vi "libssh2_userauth_password_ex.vi"(7 "passwd_change_cb":u64, 8 "error in (no error)":errorcluster, 9 "password":string, 10 "username":string, 11 "session":T1) -> (0 "error out":errorcluster)   [LabVIEW 2017, in "libssh2.lvlib"]
doc: "Authenticate a session using a password with a custom password change callback."
uses:
  libssh2.lvlib
  Session Refnum.ctl
  Not A Session.vi
  <vilib>/Utility/error.llb/Error Cluster From Error Code.vi
  Global Settings.vi
  Read Session Refnum.vi
  <vilib>/Utility/semaphor.llb/Acquire Semaphore.vi
  <vilib>/Utility/semaphor.llb/Release Semaphore.vi
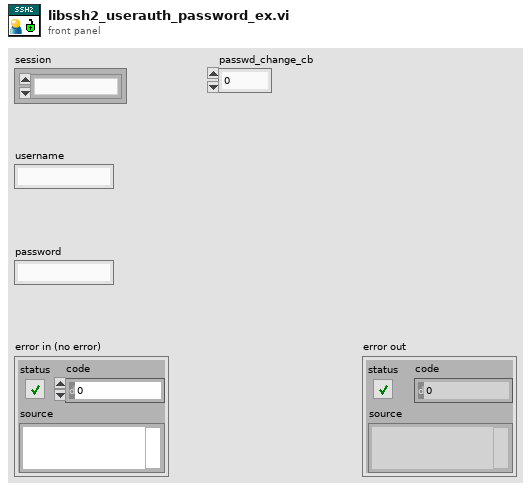
[diagram p1: front panel]
types:
  T1 = typedef "libssh2.lvlib/Session Refnum.ctl" = refnum<k1>
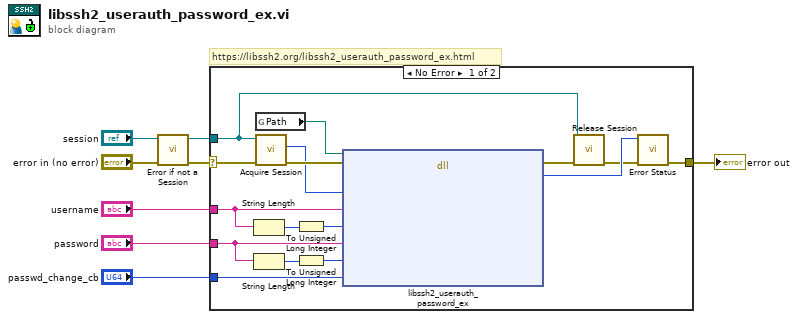
[diagram p0: block diagram]
diagram:
  # "https://libssh2.org/libssh2_userauth_password_ex.html"
  n1 = call "Error if not a Session.vi"("error in (no error)"="error in (no error)", "session"="session") -> ("error out"=w3:errorcluster, "session out"=w1:T1)  [unwired: 8 in]
  n2 = case shown="No Error" w3 {
    selector: w3 -> [w21 w25]
    tunnel: "username" -> [w24 _]
    tunnel: "password" -> [w23 _]
    tunnel: "passwd_change_cb" -> [w22 _]
    tunnel: [w20 w25] -> w5
    tunnel: w1 -> [w9 _]
    frame No Error {
      n3 = String Length(string=w24) -> (length=w15:i32)
      n4 = String Length(string=w23) -> (length=w16:i32)
      n5 = global read "Global Settings.vi" "Path"() -> (w12:path)
      n6 = call "Acquire Session.vi"("error in (no error)"=w21, "session"=w9) -> ("error out"=w14:errorcluster, "LIBSSH2_SESSION*"=w13:u64)  [unwired: 7 in, 1 out]
      n7 = To Unsigned Long Integer(number=w15) -> (unsigned 32bit integer=w19:u32)
      n8 = To Unsigned Long Integer(number=w16) -> (unsigned 32bit integer=w18:u32)
      n9 = dll-call lib="?" fn="libssh2_userauth_password_ex"(path in=w12, error in=w14, "session"=w13, "username"=w24, "username_len"=w19, "password"=w23, "password_len"=w18, "passwd_change_cb"=w22) -> (error out=w17:errorcluster, "return value"=w11:i32)  [unwired: 7 in, 1 out]
      n10 = call "Release Session.vi"("error in (no error)"=w17, "session"=w9) -> ("error out"=w10:errorcluster)  [unwired: 9 in]
      n11 = call "Error Status.vi"("error in (no error)"=w10, "return value"=w11) -> ("error out"=w20:errorcluster)  [unwired: 8 in, 1 out]
    }
    frame Error {
    }
  }
  "error out" <- w5
